vi "Cleanup.vi"(8 "error in (no error)":errorcluster, 11 "DeviceDetailPanel in":refnum<class "DeviceDetailPanel.lvclass">) -> (0 "error out":errorcluster)   [LabVIEW 2020, in "PicoG-App.lvlib" / "DeviceDetailPanel.lvclass"]
uses:
  DeviceDetailPanel.lvclass
  DeviceDetailPanel.lvclass/DeviceDetailPanel.ctl
  <vilib>/IlluminatedG/IG OOPanel/OOPanel/Panel/Panel.lvclass
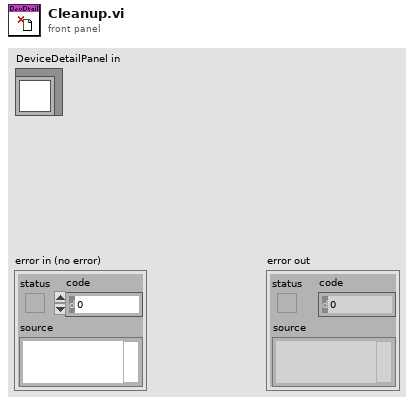
[diagram p1: front panel]
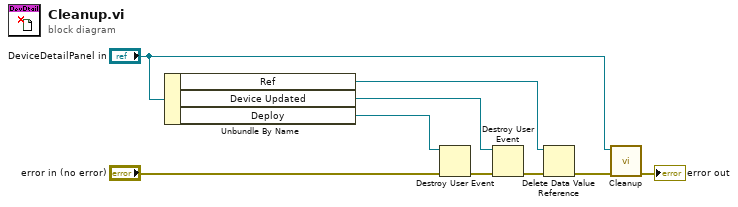
[diagram p0: block diagram]
diagram:
  n1 = Unbundle By Name("DeviceDetailPanel in") -> ("Ref"=w5:refnum<data-value>, "Device Updated"=w7:refnum<user-event>, "Deploy"=w1:refnum<user-event>)
  n2 = Destroy User Event(user event=w1, error in="error in (no error)") -> (error out=w3:errorcluster)
  n3 = Destroy User Event(user event=w7, error in=w3) -> (error out=w6:errorcluster)
  n4 = Delete Data Value Reference(data value reference=w5, error in=w6) -> (error out=w4:errorcluster)  [unwired: 1 out]
  n5 = call-parent "Cleanup.vi"("error in (no error)"=w4, "Panel in"="DeviceDetailPanel in") -> ("error out"=→"error out":errorcluster)  [unwired: 9 in]
